vi "Parse Mark Harmonic.vi"(8 "error in (no error)":errorcluster caption="에러 입력(에러 없음)", 10 "JSON string":string, 11 "Instrument Manager 입력":refnum<class "Instrument Manager.lvclass">) -> (0 "error out":errorcluster caption="에러 출력", 1 "Fundamental Frequency":dbl, 2 "Mark Harmonic Param":T1, 3 "Instrument Manager 출력":refnum<class "Instrument Manager.lvclass">)   [LabVIEW 2023, in "Instrument Manager.lvclass"]
uses:
  Instrument Manager.lvclass
  Instrument Manager.lvclass/Instrument Manager.ctl
  Param Definition/Mark Harmonic Param.ctl
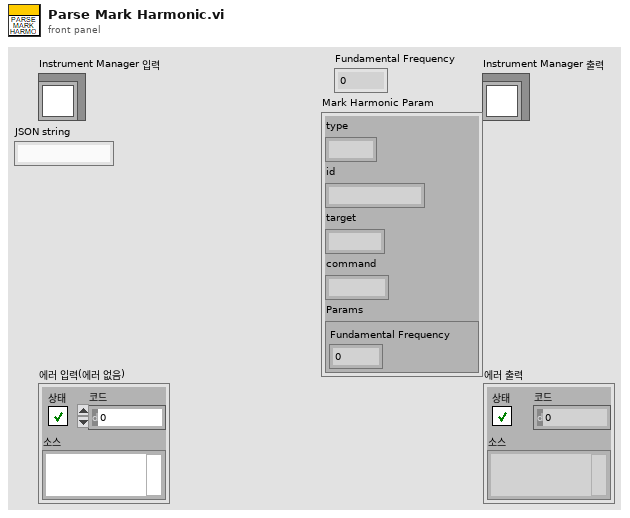
[diagram p1: front panel]
types:
  T1 = typedef "Instrument Manager.lvclass/Mark Harmonic Param.ctl" = cluster{"type":string, "id":string, "target":string, "command":string, "Params":cluster{"Fundamental Frequency":dbl}}
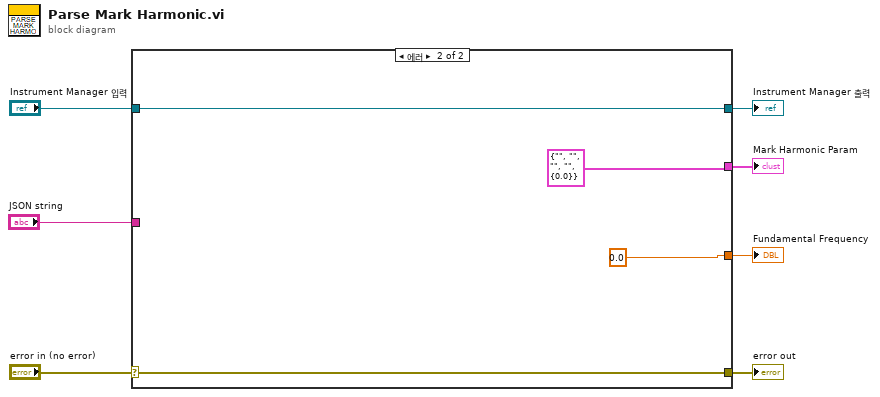
[diagram p0: block diagram]
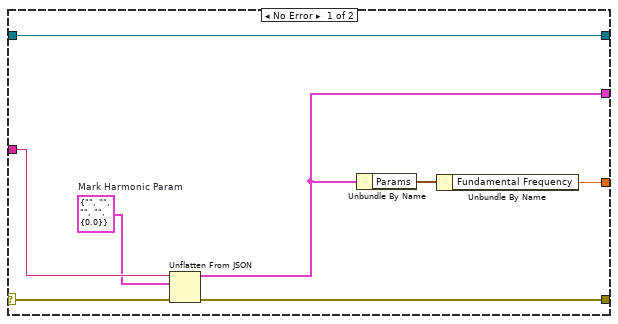
[diagram p2: hidden frame]
diagram:
  n1 = case shown="에러" "error in (no error)" {
    selector: "error in (no error)" -> [w14 w19]
    tunnel: [w11 w19] -> w6
    tunnel: [w15 w18] -> w4
    tunnel: "Instrument Manager 입력" -> [w15 w18]
    tunnel: "JSON string" -> [w13 _]
    tunnel: [w9 0.0 ("Fundamental Frequency")] -> w2
    tunnel: [w8 T1 {"type"="", "id"="", "target"="", "command"="", "Params"={"Fundamental Frequency"=0.0}} ("Mark Harmonic Param")] -> w1
    frame No Error {
      w12 = T1 {"type"="", "id"="", "target"="", "command"="", "Params"={"Fundamental Frequency"=0.0}}  # Mark Harmonic Param
      n2 = Unflatten From JSON(JSON string=w13, type and defaults=w12, error in (no error)=w14) -> (value=w8:T1, error out=w11:errorcluster)  [unwired: 4 in]
      n3 = Unbundle By Name(w8) -> ("Params"=w10:cluster{"Fundamental Frequency":dbl})
      n4 = Unbundle By Name(w10) -> ("Fundamental Frequency"=w9:dbl)
    }
    frame Error {
    }
  }
  "error out" <- w6
  "Instrument Manager 출력" <- w4
  "Fundamental Frequency" <- w2
  "Mark Harmonic Param" <- w1
